vi "Get lv_python_grpc_webui_demo_v1_ChamberStatus.vi"(8 "error in (no error)":errorcluster, 11 "gRPCid":T1) -> (0 "error out":errorcluster, 2 "package_templatemessage":T2, 3 "gRPCid out":T1)   [LabVIEW 2020, in "thermal-chamber-controller_server.lvlib"]
uses:
  thermal-chamber-controller_server.lvlib
  lv_python_grpc_webui_demo_v1_ChamberStatus.ctl
  lv_python_grpc_webui_demo_v1_HeaterState.ctl
  <vilib>/gRPC/LabVIEW gRPC Library/Shared/grpcId.ctl
  lv_python_grpc_webui_demo_v1_ChamberStatus_Flat.ctl
  2ed25e12-861d-4677-8ead-ace2906b2041.vi
  <vilib>/gRPC/LabVIEW gRPC Library/Shared/TranslateGrpcError.vi
  <vilib>/gRPC/LabVIEW gRPC Library/Server API/Server/Get Server DLL Path.vi
  <vilib>/Utility/error.llb/Error Cluster From Error Code.vi
  <vilib>/gRPC/LabVIEW gRPC Library/grpc-lvsupport-release.lvlib
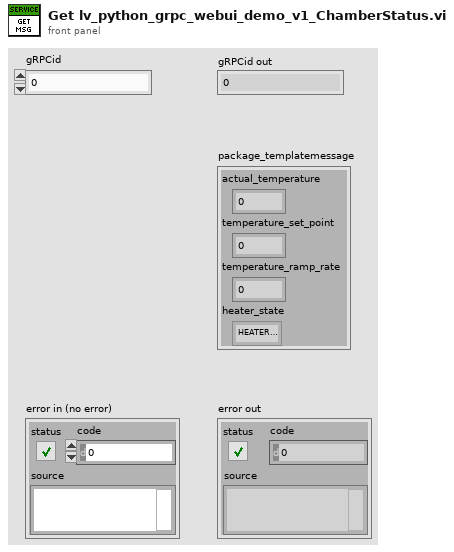
[diagram p1: front panel]
types:
  T1 = typedef "grpc-lvsupport-release.lvlib/grpcId.ctl" = u64
  T2 = typedef "thermal-chamber-controller_server.lvlib/lv_python_grpc_webui_demo_v1_ChamberStatus.ctl" = cluster{"actual_temperature":dbl, "temperature_set_point":dbl, "temperature_ramp_rate":dbl, "heater_state":T3}
  T3 = typedef "thermal-chamber-controller_server.lvlib/lv_python_grpc_webui_demo_v1_HeaterState.ctl" = enum32{"HEATER_ENABLED", "HEATER_DISABLED"}
  T4 = typedef "thermal-chamber-controller_server.lvlib/lv_python_grpc_webui_demo_v1_ChamberStatus_Flat.ctl" = cluster{"actual_temperature":dbl, "temperature_set_point":dbl, "temperature_ramp_rate":dbl, "heater_state":T3}
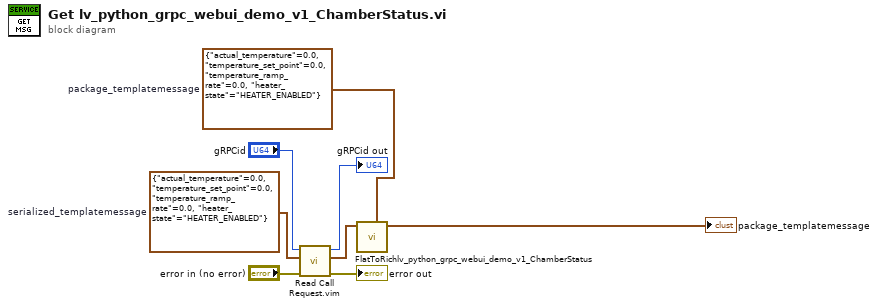
[diagram p0: block diagram]
diagram:
  w6 = T4 {"actual_temperature"=0.0, "temperature_set_point"=0.0, "temperature_ramp_rate"=0.0, "heater_state"=enum."HEATER_ENABLED"}  # serialized_templatemessage
  w5 = T2 {"actual_temperature"=0.0, "temperature_set_point"=0.0, "temperature_ramp_rate"=0.0, "heater_state"=enum."HEATER_ENABLED"}  # package_templatemessage
  n1 = call "Read Call Request.vim"("error in"="error in (no error)", "Request Type"=w6, "gRPCid in"="gRPCid") -> ("error out"=→"error out":errorcluster, "Request Data"=w4:T4, "gRPCid out"=→"gRPCid out":T1)  [unwired: 6 in]
  n2 = call "FlatToRichlv_python_grpc_webui_demo_v1_ChamberStatus.vi"("OutputClusterType"=w5, "InputCluster"=w4) -> ("OutputCluster"=→"package_templatemessage":T2)  [unwired: 9 in]
